vi "Get Argument.vi"(9 "error in (no error)":errorcluster, 11 "argument":string) -> (1 "error out":errorcluster, 2 "found?":bool, 3 "argument data":string)   [LabVIEW 2019, in "Error Generation.lvlib"]
doc: "Get the data for the argument. The argument name is case insensitive!\nIf argument is not found data is empty.\n- - -\nCopyright (c) 2023, Merecs Engineering GmbH"
uses:
  Error Generation.lvlib
panel:
  # "Connector Pane"
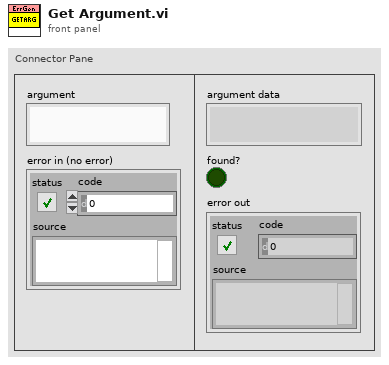
[diagram p1: front panel]
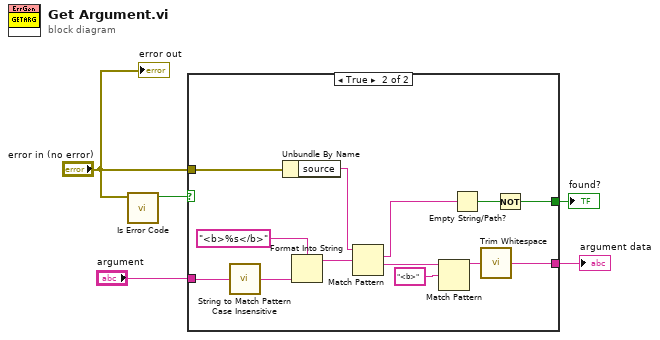
[diagram p0: block diagram]
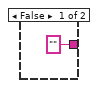
[diagram p2: hidden frame]
diagram:
  n1 = call "Is Error Code.vi"("error in (no error)"="error in (no error)") -> ("Code!=0"=w2:bool)  [unwired: 5 in, 1 out]
  n2 = case shown="True" w2 {
    tunnel: "argument" -> [_ w8]
    tunnel: ["" ("trimmed string") w16] -> w4
    tunnel: "error in (no error)" -> [_ w12]
    tunnel: [_ w9] -> w1
    frame False {
    }
    frame True {
      n3 = call "String to Match Pattern Case Insensitive.vi"("Input String"=w8) -> ("String"=w7:string)
      n4 = Unbundle By Name(w12) -> ("source"=w13:string)
      n5 = Format Into String(format string="<b>%s</b>", w7) -> (resulting string=w14:string)  [unwired: 2 in, 1 out]
      n6 = Match Pattern(string=w13, regular expression=w14) -> (match substring=w11:string, after substring=w17:string)  [unwired: 1 in, 2 out]
      n7 = Match Pattern(string=w17, regular expression="<b>") -> (before substring=w18:string)  [unwired: 1 in, 3 out]
      n8 = Empty String/Path?(string/path=w11) -> (empty?=w10:bool)
      n9 = call <vilib>:"Trim Whitespace.vi"("string"=w18) -> ("trimmed string"=w16:string)  [unwired: 1 in]
      n10 = Not(x=w10) -> (.not. x?=w9:bool)
    }
  }
  "argument data" <- w4
  "found?" <- w1
  "error out" <- "error in (no error)"
